vi "ReleaseDC Wrapper Template.vi"(0 "hWnd":u64, 5 "hDC":u64, 11 "error in":errorcluster) -> (4 "return value":i32, 15 "error out":errorcluster)   [LabVIEW 2020]
doc: "Releases a device context obtained with user32 GetDC.vi, through user32.dll ReleaseDC (stdcall, called in any thread). hWnd must be the window that was passed to GetDC (0 for the screen). return value is 1 when the DC was released, 0 when it was not. When error in carries an error the DLL is not called. Generated by scripts\\Build Win32 Wrappers.vi - do not edit by hand, rebuild it."
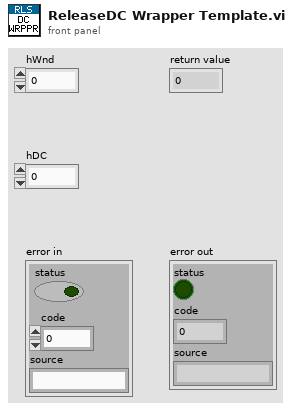
[diagram p1: front panel]
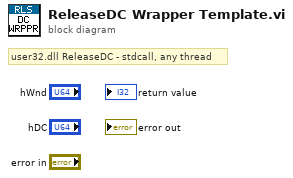
[diagram p0: block diagram]
diagram:
  # "user32.dll ReleaseDC - stdcall, any thread"
